vi "LTE set BandWidth.vi"(8 "error in (no error)":errorcluster caption="에러 입력(에러 없음)", 10 "BandWidth":T1, 11 "Instrument Manager 입력":refnum<class "Instrument Manager.lvclass">) -> (0 "error out":errorcluster caption="에러 출력", 3 "Instrument Manager 출력":refnum<class "Instrument Manager.lvclass">)   [LabVIEW 2023, in "Instrument Manager.lvclass"]
uses:
  Instrument Manager.lvclass
  Instrument Manager.lvclass/Instrument Manager.ctl
  Module/ANRITSU Call Box/Interface Class/Anritsu Call Box.lvclass
  Module/ANRITSU Call Box/Type Definition/LTE Channel Type.ctl
  Module/ANRITSU Call Box/ANRITSU Call Box.lvlib
  Module/ANRITSU Call Box/Type Definition/LTE Supported BandWidth.ctl
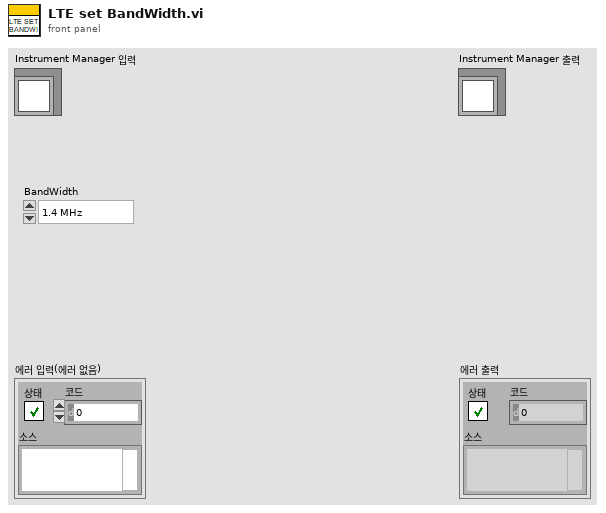
[diagram p1: front panel]
types:
  T1 = typedef "ANRITSU Call Box.lvlib/LTE Supported BandWidth.ctl" = enum16{"1.4 MHz", "3 MHz", "5 MHz", "10 MHz", "15 MHz", "20 MHz"}
  T2 = typedef "ANRITSU Call Box.lvlib/LTE Channel Type.ctl" = enum16{"PCC", "SCC1", "SCC2", "SCC3"}
  T3 = cluster{"Anritsu Call Box":refnum<class "Anritsu Call Box.lvclass">, "Spectrum Analyzer":refnum<class "Interface_Spectrum.lvclass">, "RF Switch Box":refnum<class "RF Filter Box.lvclass">, "Turn Table":refnum<class "Interface - Turn Table.lvclass">, "Mast":refnum<class "Interface - Mast.lvclass">, "3D Controller":refnum<class "Interface_3D Controller.lvclass">}
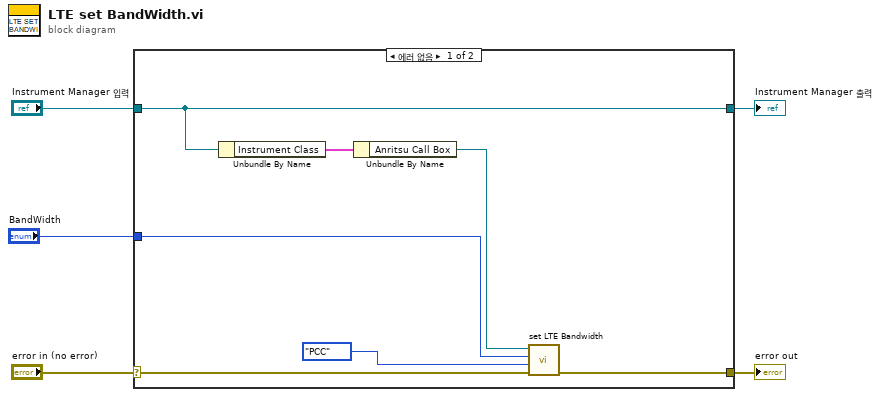
[diagram p0: block diagram]
diagram:
  n1 = case shown="에러 없음" "error in (no error)" {
    selector: "error in (no error)" -> [w12 w14]
    tunnel: [w11 w14] -> w4
    tunnel: [w10 w13] -> w2
    tunnel: "Instrument Manager 입력" -> [w10 w13]
    tunnel: "BandWidth" -> [w6 _]
    frame No Error {
      n2 = Unbundle By Name(w10) -> ("Instrument Class"=w9:T3)
      n3 = Unbundle By Name(w9) -> ("Anritsu Call Box"=w8:refnum<class "Anritsu Call Box.lvclass">)
      n4 = call-dynamic "set LTE Bandwidth.vi"("error in (no error)"=w12, "LTE Channel Type"=LTE_Channel_Type."PCC", "BandWidth"=w6, "Anritsu Call Box in"=w8) -> ("error out"=w11:errorcluster)  [unwired: 6 in, 1 out]
    }
    frame Error {
    }
  }
  "error out" <- w4
  "Instrument Manager 출력" <- w2
